vi "JYSp.vi"() -> ()   [LabVIEW 2015]
uses:
  <vilib>/Utility/file.llb/Write Delimited Spreadsheet (I64).vi
panel:
  out "画图横轴":i32[][](array[numeric])
  out "Spectrum":cluster{"Y":dbl[], "Y":dbl[]}[](graph)
  out "Data":i32[](array[numeric])
  out "Intensity Graph":dbl[][](graph)
  out "最终存储路径":path
  in  "Move To\nTarget Positions":bool
  in  "Target\nFront Entrance":dbl=1.0
  in  "Entrance Mirror":u16(ring)=2 caption="Target Position\nEntrance Mirror" items=["Front"=2, "Side"=3]
  in  "Exit Mirror":u16(ring)=3 caption="Target Position Exit Mirror" items=["Front"=2, "Side"=3]
  in  "Target WL":dbl=710.0
  out "Front Entrance":dbl
  out "Units 2":string="mm"
  out "error out":errorcluster
  out "Entrance Mirror\nPosition":i32(ring)=2 items=["EntranceMirror", "ExitMirror", "Front", "Side"]
  out "Exit Mirror\nPosition":i32(ring)=2 items=["EntranceMirror", "ExitMirror", "Front", "Side"]
  out "Current WL":dbl=897.9988
  out "Units":string="nm"
  out "Current Grating":dbl=1200.0
  out "Grating Index":i32=1
  out "Current Description":string="1" caption="Description"
  in  "Target Grating":string(combo)="2"
  out "Gratings":dbl[](array[numeric])=[1200.0, 300.0]
  in  "Force\nInitialization":bool
  out "Initialized JY":bool=TRUE
  in  "Connect":bool
  in  "Mono ID":string(combo)="Mono1"
  out "Current UniqueID":string="Mono4"
  in  "Constante de condition\n(Voir l'aide contextuelle)":bool
  out "trigAddress":i32
  in  "Commande tab":T1(tab)
  in  "Area Number to Display":i32
  in  "Reformat":bool
  in  "GAIN":u16(ring) caption="Device Name" items=["High Light", "Best Dynamic Range", "High Sensitivity"]
  in  "ADC":u16(ring) caption="Device Name" items=["20 kHz       ", " 1 MHz       ", " 1 MHz Ultra "]
  in  "Number of Areas :":u16=1 min=1 step=1
  in  "Integration time (ms) :":i16=500
  out "Uniques ID":u16(ring) items=["CCD1", "CCD2"]
  in  "Device Name":u16(ring) items=["Synapse CCD (Lateral)", "Synapse_IGA (Axial)"]
  in  "Signal type :":enum16{"TTL Rising Edge", "TTL Falling Edge"}(ring)=enum."TTL Falling Edge"
  in  "Trigger Type :":u16(ring) items=["On Start"=1, "Per Acquisition"=2]
  in  "trigSigTypeString":string
  in  "trigEventString":string
  in  "Enable InputTriggers :":bool
  in  "Number of Cleans":i32=1
  in  "MultiAcqShutterMode":i32(ring)=3 items=["Open For All Spectra"=1, "Open for Each Spectrum"=3]
  in  "Accumulations:":u16=10 min=1 step=1
  in  "Multi Accumulation mode:":bool
  out "Y Pixels:":i32=256
  out "DataSize":i32=1024
  out "X Pixels:":i32=1024
  out "Firmware\nVersion":string="V1.20 CCD_4000"
  out "Acq Time(ms)":u32=3401
  out "Gain Number":i32[](array[numeric])=[10, 11, 12, 13, 8, 2]
  out "ADC Number":i32[](array[numeric])=[0, 1, 2, 3, 4]
  out "initialized ?":bool=TRUE
  in  "Continuous":bool
  in  "CCD Busy":bool
  in  "ShutterOpen":bool=TRUE caption="Shutter enable"
  out "temp graph":dbl(graph)=-134.538067
  in  "Temperature":bool
  out "areas :":i32[][](array[numeric])=[[1], [1], [1], [1024], [256], [1], [256]]
  in  "Acquire":bool
  in  "Setup":bool
  in  "Close":bool=TRUE
  out "indicator":string="Ready !"
  in  "initialize":bool
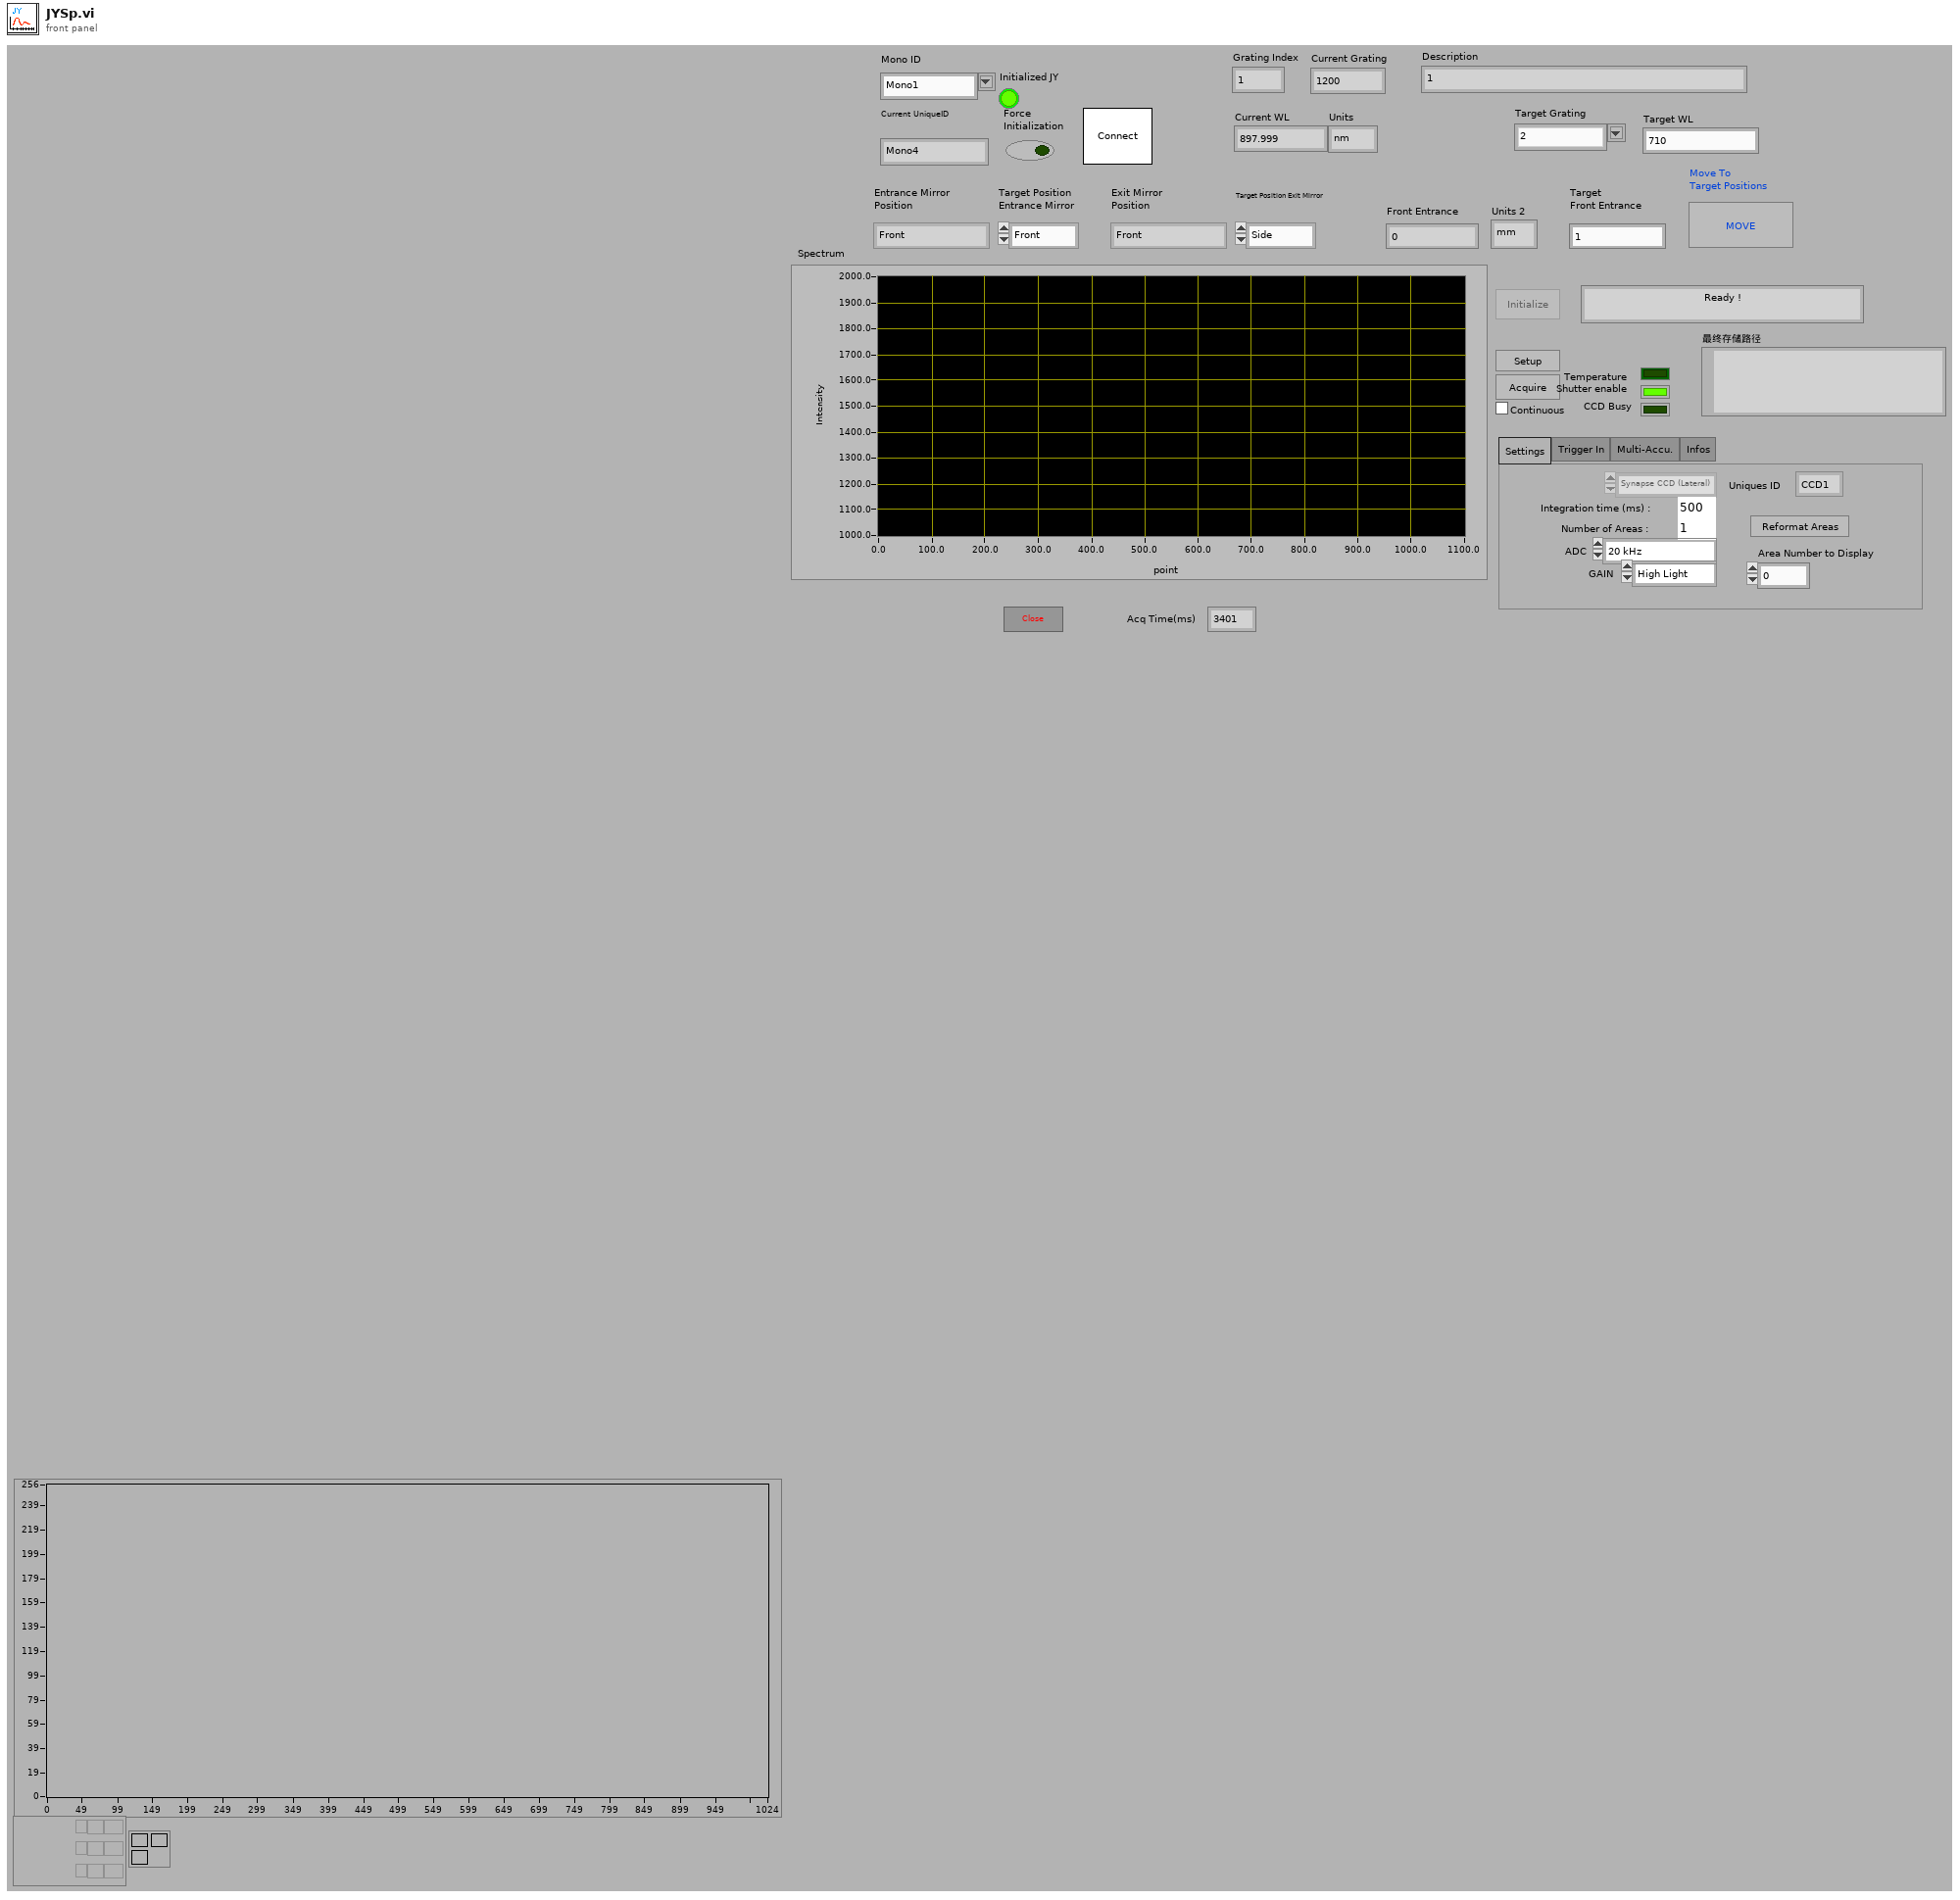
[diagram p1: front panel]
types:
  T1 = enum32{"Settings", "Trigger In", "Multi-Accu.", "Infos"}
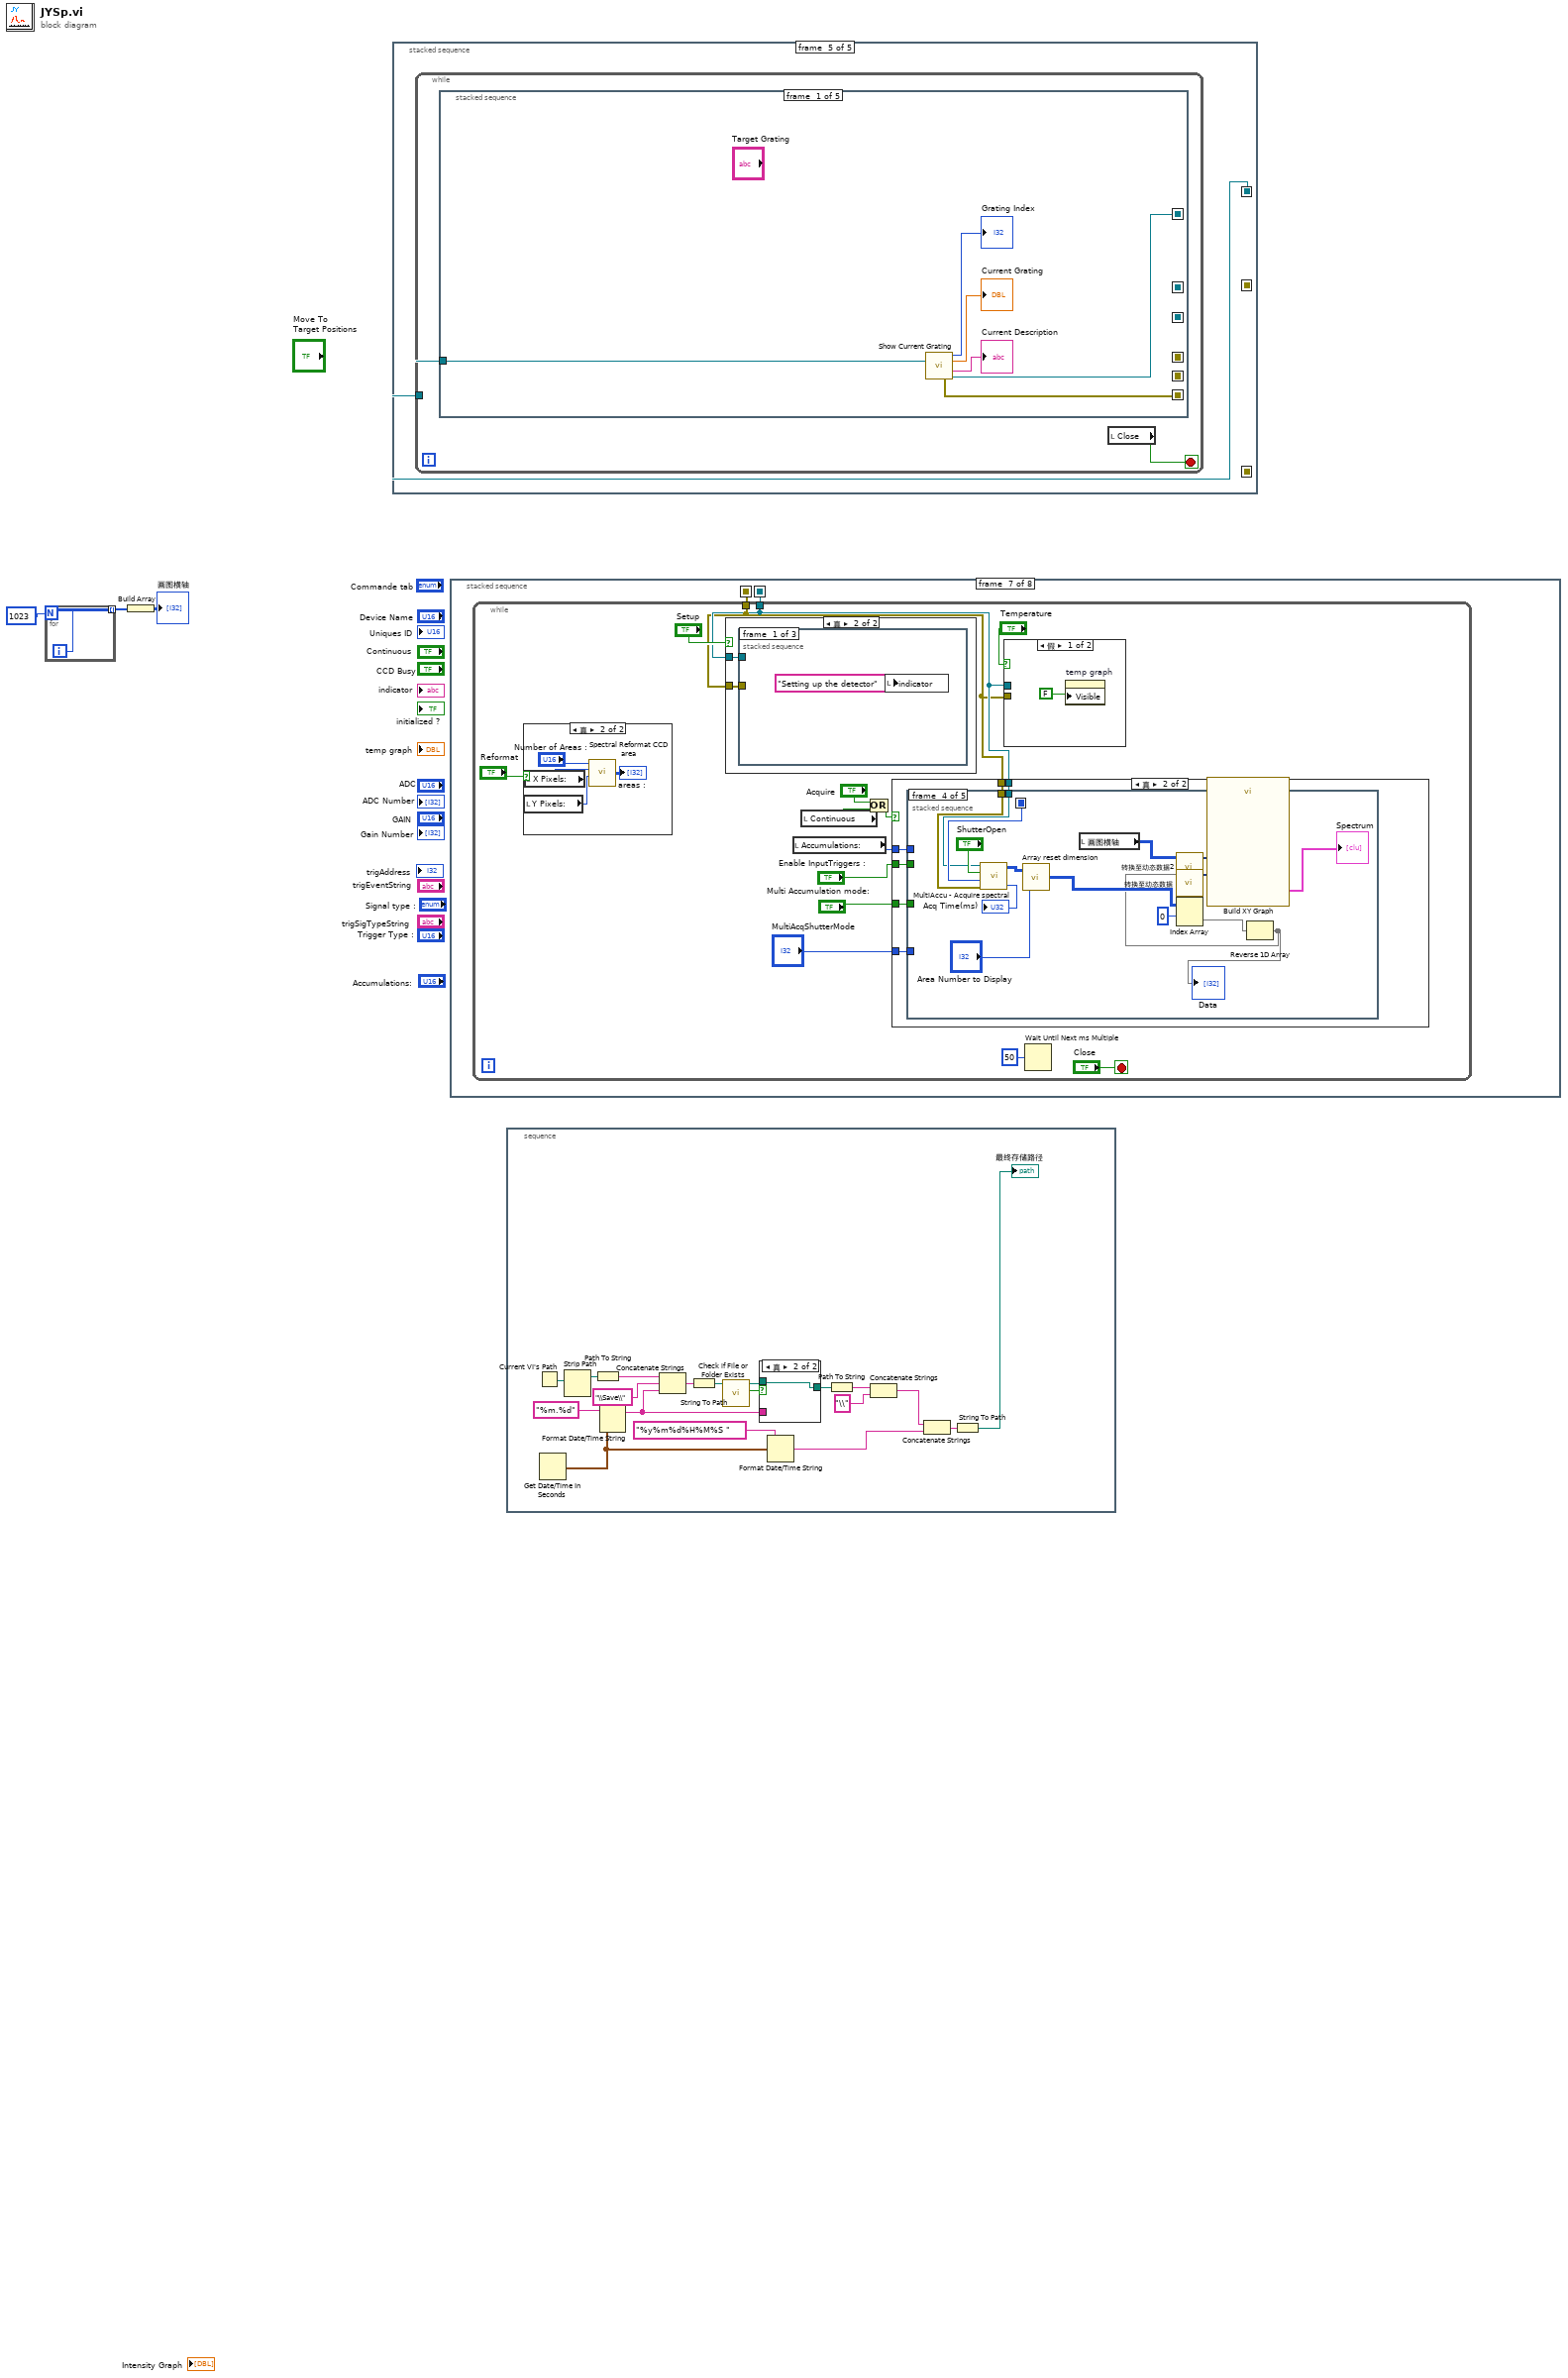
[diagram p0: block diagram]
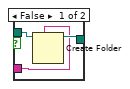
[diagram p2: hidden frame]
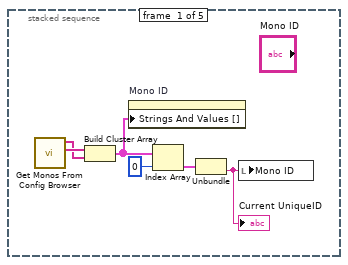
[diagram p3: hidden frame]
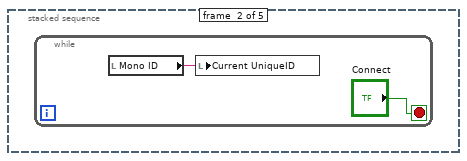
[diagram p4: hidden frame]
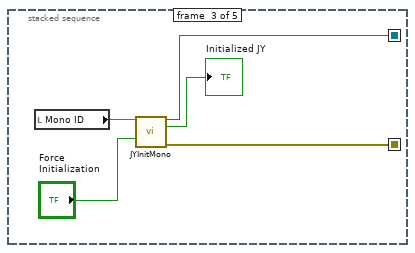
[diagram p5: hidden frame]
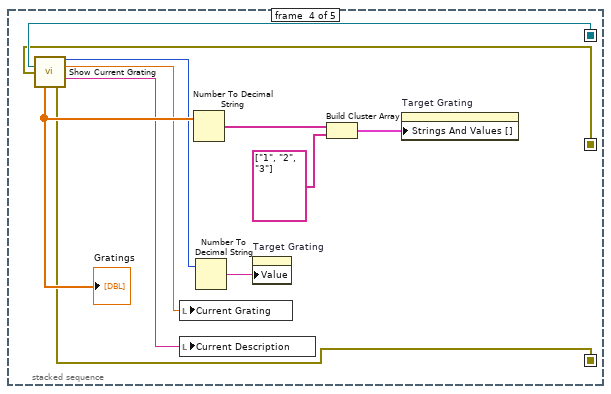
[diagram p6: hidden frame]
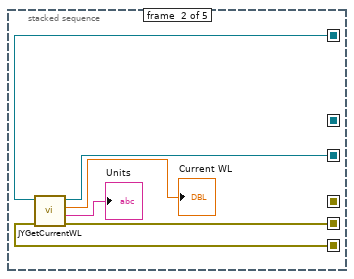
[diagram p7: hidden frame]
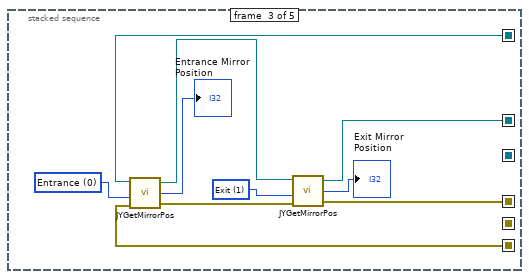
[diagram p8: hidden frame]
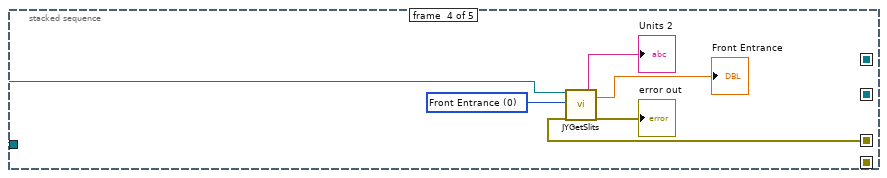
[diagram p9: hidden frame]
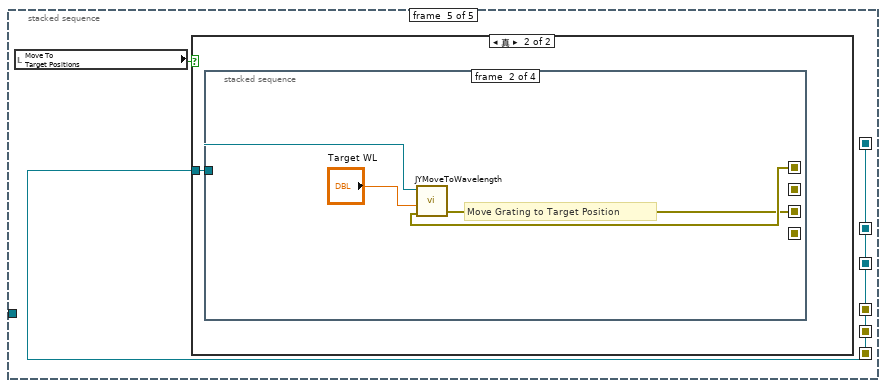
[diagram p10: hidden frame]
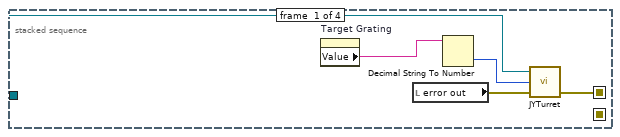
[diagram p12: hidden frame]
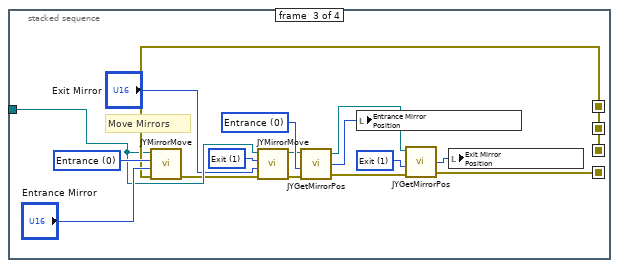
[diagram p13: hidden frame]
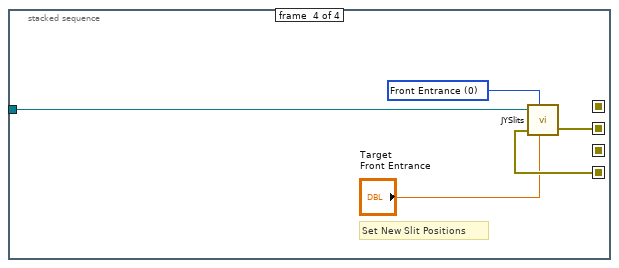
[diagram p14: hidden frame]
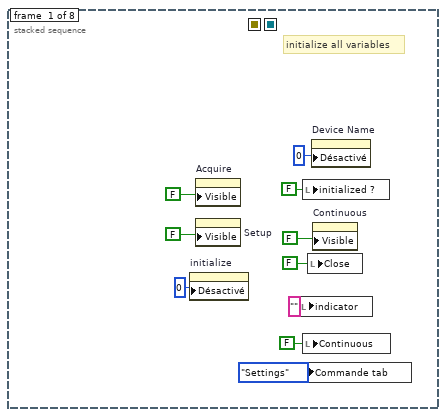
[diagram p15: hidden frame]
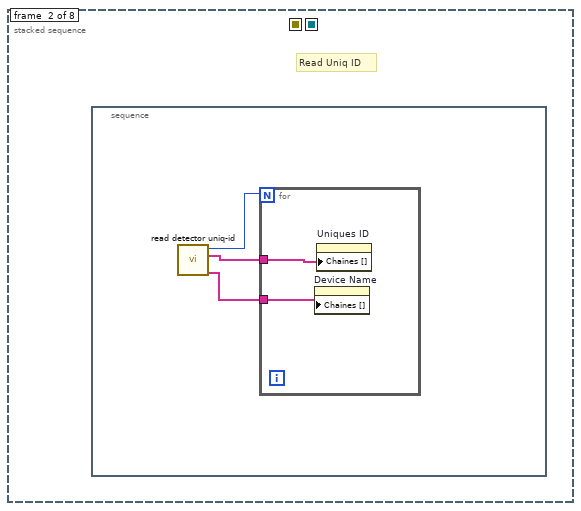
[diagram p16: hidden frame]
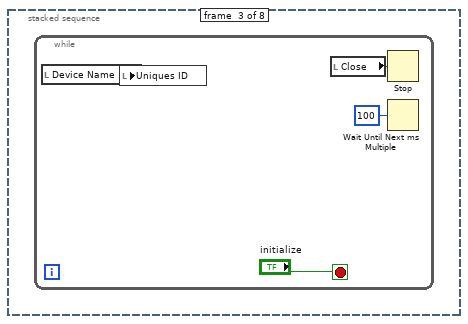
[diagram p17: hidden frame]
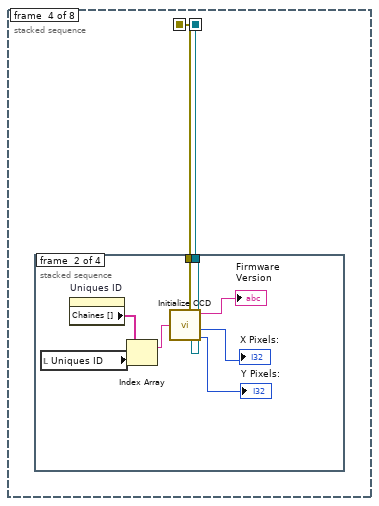
[diagram p18: hidden frame]
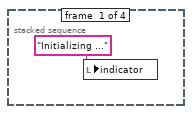
[diagram p19: hidden frame]
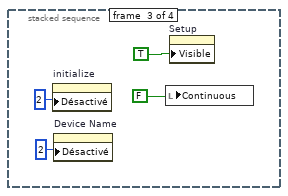
[diagram p20: hidden frame]
diagram:
  n1 = for {
    N: 1023 -> [_]
    tunnel: [w4] -> w3 mode=indexing
    i -> [w4]
  }
  n2 = Build Array(w3) -> (→"画图横轴":i32[][])
  n3 = stacked-sequence {
    seq-local: [_ _ w14 _ _] -> [_ _ _ w24 w29]
    seq-local: [_ _ w13 _ _] -> [_ _ _ w23 _]
    seq-local: [_ _ _ w22 _] -> [_ _ _ _ _]
    frame #0 {
      n4 = call "Get Monos From Config Browser.vi"() -> ("UniqueIDs"=w9:string[], "Mono ID"=w10:string[])  [unwired: 3 in, 1 out]
      n5 = Build Cluster Array(w10, w9) -> (w7:cluster{"String":string, "String":string}[])
      n6 = property on="Mono ID" class="CmbBox"("Strings And Values []"=w7) -> ()  [unwired: 2 in, 2 out]
      n7 = Index Array(array=w7, index=0) -> (element=w8:cluster{"String":string, "String":string})
      n8 = Unbundle(w8) -> ("String"=w5:string)  [unwired: 1 out]
      "Current UniqueID" <- w5
      n9 = local write "Mono ID"(w5) -> ()
    }
    frame #1 {
      n10 = while {
        stop <- "Connect" stop-if-true
        n11 = local read "Mono ID"() -> (w11:string)
        n12 = local write "Current UniqueID"(w11) -> ()
      }
    }
    frame #2 {
      n13 = local read "Mono ID"() -> (w16:string)
      n14 = call "JYInitMono.vi"("Unique ID"=w16, "Force Init"="Force\nInitialization") -> ("Refnum out"=w14:refnum<k7>, "Initialized"=→"Initialized JY":bool, "error out"=w13:errorcluster)  [unwired: 9 in, 2 out]
    }
    frame #3 {
      n15 = call "Show Current Grating.vi"("Refnum in"=w24, "error in (no error)"=w23) -> ("Gratings"=w25:dbl[], "Grating Index"=w19:i32, "Current Grating"=w21:dbl, "Current Description"=w18:string, "error out"=w22:errorcluster)  [unwired: 5 in, 4 out]
      "Gratings" <- w25
      n16 = local write "Current Grating"(w21) -> ()
      n17 = local write "Current Description"(w18) -> ()
      n18 = Number To Decimal String(number=w25) -> (decimal integer string=w27:string[])  [unwired: 1 in]
      n19 = Number To Decimal String(number=w19) -> (decimal integer string=w20:string)  [unwired: 1 in]
      n20 = property on="Target Grating" class="CmbBox"("Value"=w20) -> ()  [unwired: 2 in, 2 out]
      n21 = Build Cluster Array(w27, string[] ["1", "2", "3"]) -> (w28:cluster{"Numeric":string, string}[])
      n22 = property on="Target Grating" class="CmbBox"("Strings And Values []"=w28) -> ()  [unwired: 2 in, 2 out]
    }
    frame #4 {
      n23 = while {
        tunnel: w29 -> [w31]
        stop <- w30 stop-if-true
        n24 = stacked-sequence {
          seq-local: [w35 _ _ _ _] -> [_ w42 w53 _ w60]
          seq-local: [w34 _ _ _ _] -> [_ w41 w52 _ _]
          seq-local: [_ w40 _ _ _] -> [_ _ _ _ _]
          seq-local: [_ w39 _ _ _] -> [_ _ _ _ _]
          seq-local: [_ _ w45 _ _] -> [_ _ _ _ _]
          seq-local: [_ _ w44 _ _] -> [_ _ _ w55 _]
          tunnel: w31 -> [w33 _ _ w56 _]
          frame #0 {
            n25 = call "Show Current Grating.vi"("Refnum in"=w33) -> ("Grating Index"=→"Grating Index":i32, "Current Grating"=→"Current Grating":dbl, "Current Description"=→"Current Description":string, "error out"=w34:errorcluster, "JYMONOLib.IJYMonoReqd"=w35:refnum<k7>)  [unwired: 6 in, 4 out]
          }
          frame #1 {
            n26 = call "JYGetCurrentWL.vi"("error in (no error)"=w41, "JYMONOLib.IJYMonoReqd"=w42) -> ("error out"=w39:errorcluster, "Units"=→"Units":string, "Current WL"=→"Current WL":dbl, "JYMONOLib.IJYMonoReqd 2"=w40:refnum<k7>)  [unwired: 6 in]
          }
          frame #2 {
            w50 = u16 1 items=["Entrance", "Exit"] ("Mirror Number")
            w51 = u16 0 items=["Entrance", "Exit"] ("Mirror Number")
            n27 = call "JYGetMirrorPos.vi"("error in (no error)"=w52, "Mirror"=w51, "Refnum In"=w53) -> ("error out"=w48:errorcluster, "Current Mirror Position"=→"Entrance Mirror\nPosition":i32, "Refnum Out"=w49:refnum<k7>)  [unwired: 1 in]
            n28 = call "JYGetMirrorPos.vi"("error in (no error)"=w48, "Mirror"=w50, "Refnum In"=w49) -> ("error out"=w44:errorcluster, "Current Mirror Position"=→"Exit Mirror\nPosition":i32, "Refnum Out"=w45:refnum<k7>)  [unwired: 1 in]
          }
          frame #3 {
            w58 = u16 0 items=["Front Entrance", "Side Entrance", "Front Exit", "Side Exit", "First Intermediate", "Second Intermediate"] ("Slit")
            n29 = call "JYGetSlits.vi"("MonoRefNum IN"=w56, "Slit"=w58, "error in (no error)"=w55) -> ("Units"=→"Units 2":string, "Slit Width"=→"Front Entrance":dbl, "error out"=→"error out":errorcluster)  [unwired: 13 in, 1 out]
          }
          frame #4 {
            n30 = local read "Move To\nTarget Positions"() -> (w61:bool)
            n31 = case shown="真" w61 {
              tunnel: w60 -> [_ w62]
              frame False {
              }
              frame True {
                n32 = stacked-sequence {
                  seq-local: [w64 _ _ _] -> [_ w70 _ _]
                  seq-local: [_ w68 _ _] -> [_ _ w85 _]
                  seq-local: [_ _ w72 _] -> [_ _ _ w91]
                  seq-local: [_ _ _ w88] -> [_ _ _ _]
                  tunnel: w62 -> [w66 w69 w83 w92]
                  frame #0 {
                    n33 = property on="Target Grating" class="CmbBox"() -> ("Value"=w63:string)  [unwired: 2 in, 2 out]
                    n34 = local read "error out"() -> (w65:errorcluster)
                    n35 = Decimal String To Number(string=w63) -> (number=w67:i32)  [unwired: 2 in, 1 out]
                    n36 = call "JYTurret.vi"("error in (no error)"=w65, "Grating Index"=w67, "JYMONOLib.IJYMonoReqd"=w66) -> ("error out"=w64:errorcluster)  [unwired: 2 out]
                  }
                  frame #1 {
                    # "Move Grating to Target Position"
                    n37 = call "JYMoveToWavelength.vi"("error in (no error)"=w70, "Target WL"="Target WL", "RefNum In"=w69) -> ("error out"=w68:errorcluster)  [unwired: 1 in, 2 out]
                  }
                  frame #2 {
                    w78 = u16 1 items=["Entrance", "Exit"] ("Mirror Number")
                    w77 = u16 0 items=["Entrance", "Exit"] ("Mirror Number")
                    w84 = u16 1 items=["Entrance", "Exit", "Front", "Side"] ("Mirror Number")
                    w87 = u16 0 items=["Entrance", "Exit", "Front", "Side"] ("Mirror Number")
                    # "Move Mirrors"
                    n38 = call "JYMirrorMove.vi"("error in (no error)"=w85, "Mirror Position"="Entrance Mirror", "Mirror Number"=w87, "RefNum In"=w83) -> ("error out"=w82:errorcluster)  [unwired: 6 in, 1 out]
                    n39 = call "JYMirrorMove.vi"("error in (no error)"=w82, "Mirror Position"="Exit Mirror", "Mirror Number"=w84, "RefNum In"=w83) -> ("error out"=w75:errorcluster, "MonoRefNum Out"=w76:refnum<k7>)  [unwired: 6 in]
                    n40 = call "JYGetMirrorPos.vi"("error in (no error)"=w75, "Mirror"=w77, "Refnum In"=w76) -> ("error out"=w80:errorcluster, "Current Mirror Position"=w74:i32, "Refnum Out"=w79:refnum<k7>)  [unwired: 1 in]
                    n41 = local write "Entrance Mirror\nPosition"(w74) -> ()
                    n42 = call "JYGetMirrorPos.vi"("error in (no error)"=w80, "Mirror"=w78, "Refnum In"=w79) -> ("error out"=w72:errorcluster, "Current Mirror Position"=w73:i32)  [unwired: 1 in, 1 out]
                    n43 = local write "Exit Mirror\nPosition"(w73) -> ()
                  }
                  frame #3 {
                    w90 = u16 0 items=["Front Entrance", "Side Entrance", "Front Exit", "Side Exit", "First Intermediate", "Second Intermediate"] ("Slit")
                    # "Set New Slit Positions"
                    n44 = call "JYSlits.vi"("JYMONOLib.IJYMonoReqd"=w92, "Slit"=w90, "error in (no error)"=w91, "Slit Width"="Target\nFront Entrance") -> ("error out"=w88:errorcluster)  [unwired: 1 in, 1 out]
                  }
                }
              }
            }
          }
        }
        n45 = local read "Close"() -> (w30:bool)
      }
    }
  }
  n46 = stacked-sequence {
    seq-local: [_ _ _ w113 _ _ _ _] -> [_ _ _ _ w131 w151 w154 w266]
    seq-local: [_ _ _ w112 _ _ _ _] -> [_ _ _ _ w132 w152 w153 w267]
    frame #0 {
      # "initialize all variables"
      n47 = property on="initialize" class="Bool"("Désactivé"=u8 0) -> ()  [unwired: 2 in, 2 out]
      n48 = property on="Acquire" class="Bool"("Visible"=FALSE) -> ()  [unwired: 2 in, 2 out]
      n49 = property on="Setup" class="Bool"("Visible"=FALSE) -> ()  [unwired: 2 in, 2 out]
      n50 = local write "indicator"("" ("indicator")) -> ()
      n51 = local write "Commande tab"(T1."Settings" ("Commande tab")) -> ()
      n52 = local write "initialized ?"(FALSE ("initialized ?")) -> ()
      n53 = local write "Continuous"(FALSE ("Continuous")) -> ()
      n54 = local write "Close"(FALSE ("Close")) -> ()
      n55 = property on="Device Name" class="Ring (严格)"("Désactivé"=u8 0) -> ()  [unwired: 2 in, 2 out]
      n56 = property on="Continuous" class="Bool (严格)"("Visible"=FALSE) -> ()  [unwired: 2 in, 2 out]
    }
    frame #1 {
      # "Read Uniq ID"
      n57 = stacked-sequence {
        frame #0 {
          n58 = call <userlib>:"read detector uniq-id.vi"() -> ("nbr of components"=w105:i32, "UniqueID"=w104:string[], "Name"=w103:string[])  [unwired: 4 out]
          n59 = for {
            N: w105 -> [_]
            tunnel: w104 -> [w107]
            tunnel: w103 -> [w106]
            n60 = property on="Device Name" class="Ring (严格)"("Chaînes []"=w106) -> ()  [unwired: 2 in, 2 out]
            n61 = property on="Uniques ID" class="Ring (严格)"("Chaînes []"=w107) -> ()  [unwired: 2 in, 2 out]
          }
        }
      }
    }
    frame #2 {
      n62 = while {
        stop <- "initialize" stop-if-true
        n63 = local read "Device Name"() -> (w110:u16)
        n64 = local write "Uniques ID"(w110) -> ()
        n65 = local read "Close"() -> (w108:bool)
        n66 = Stop(stop? (T)=w108) -> ()
        n67 = Wait Until Next ms Multiple(millisecond multiple=u32 100 ("n millisecondes")) -> ()  [unwired: 1 out]
      }
    }
    frame #3 {
      n68 = stacked-sequence {
        tunnel: [_ w120 _ _] -> w113
        tunnel: [_ w119 _ _] -> w112
        frame #0 {
          n69 = local write "indicator"("Initializing ..." ("indicator")) -> ()
        }
        frame #1 {
          n70 = local read "Uniques ID"() -> (w117:u16)
          n71 = property on="Uniques ID" class="Ring (严格)"() -> ("Chaînes []"=w118:string[])  [unwired: 2 in, 2 out]
          n72 = Index Array(array=w118, index=w117) -> (element=w116:string)
          n73 = call <userlib>:"Initialize CCD.vi"("Unique id:"=w116) -> ("activeYPixels"=→"Y Pixels:":i32, "JYCCDLib.IJYCCDReqd"=w119:refnum<k7>, "activeXPixels"=→"X Pixels:":i32, "sortie d'erreur"=w120:errorcluster, "FirmwareVersion"=→"Firmware\nVersion":string)  [unwired: 3 out]
        }
        frame #2 {
          n74 = property on="initialize" class="Bool"("Désactivé"=u8 2) -> ()  [unwired: 2 in, 2 out]
          n75 = property on="Device Name" class="Ring (严格)"("Désactivé"=u8 2) -> ()  [unwired: 2 in, 2 out]
          n76 = local write "Continuous"(FALSE ("Continuous")) -> ()
          n77 = property on="Setup" class="Bool"("Visible"=TRUE) -> ()  [unwired: 2 in, 2 out]
        }
        frame #3 {
          n78 = local write "initialized ?"(TRUE ("initialized ?")) -> ()
          n79 = local write "indicator"("Initialized !" ("indicator")) -> ()
        }
      }
    }
    frame #4 {
      # "Actually not working"
      # "Read ADC and GAIN"
      n80 = case shown="真" "Constante de condition\n(Voir l'aide contextuelle)" {
        tunnel: w132 -> [_ w142]
        tunnel: w131 -> [_ w141]
        frame False {
        }
        frame True {
          # "Read Input supported trigger"
          n81 = call <userlib>:"Trigger - Get Supported Input.vi"("JYCCDLib.IJYCCDReqd"=w142, "Error Input"=w141) -> ("trigAddress"=w136:i32, "eventPtr"=w137:i32, "trigEventString"=w140:string, "trigSigType"=w139:i32, "trigSigTypeString"=w138:string)  [unwired: 4 out]
          n82 = local write "trigSigTypeString"(w138) -> ()
          n83 = local write "trigAddress"(w136) -> ()
          n84 = local write "Trigger Type :"(w137) -> ()
          n85 = local write "trigEventString"(w140) -> ()
          n86 = local write "Signal type :"(w139) -> ()
        }
      }
      n87 = call <userlib>:"Init ADC & Gain.vi"("JYCCDLib.IJYCCDReqd"=w132, "input error"=w131) -> ("ADC Number"=w130:i32[], "ADC description"=w135:string[], "Gain Number"=w133:i32[], "Gain description"=w134:string[])
      n88 = local write "Gain Number"(w133) -> ()
      n89 = local write "ADC Number"(w130) -> ()
      n90 = stacked-sequence {
        tunnel: w135 -> [w143 _]
        tunnel: w134 -> [_ w144]
        frame #0 {
          n91 = property on="ADC" class="Ring (严格)"("Chaînes []"=w143) -> ()  [unwired: 2 in, 2 out]
        }
        frame #1 {
          n92 = property on="GAIN" class="Ring (严格)"("Chaînes []"=w144) -> ()  [unwired: 2 in, 2 out]
        }
      }
    }
    frame #5 {
      # "IS multi Accumulation Supported ?"
      n93 = call <userlib>:"MultiAccu - Is Supported.vi"("Error In"=w151, "JYCCDLib.IJYCCDReqd"=w152) -> ("IsOperatingModeSupported"=w145:bool)  [unwired: 3 out]
      n94 = Select(t=0, s=w145, f=2) -> (s? t:f=w148:i32)
      n95 = Select(t=FALSE, s=w145, f=w145) -> (s? t:f=w147:bool)
      n96 = local write "Multi Accumulation mode:"(w147) -> ()
      n97 = property on="Multi Accumulation" class="Bool (严格)"("Désactivé"=w148) -> ()  [unwired: 2 in, 2 out]
      n98 = property on="Multi Accumulation mode:" class="Bool (严格)"("Désactivé"=w148) -> ()  [unwired: 2 in, 2 out]
    }
    frame #6 {
      n99 = while {
        tunnel: w153 -> [w161]
        tunnel: w154 -> [w160]
        stop <- "Close" stop-if-true
        n100 = case shown="真" "Reformat" {
          frame False {
          }
          frame True {
            n101 = local read "Y Pixels:"() -> (w244:i32)
            n102 = local read "X Pixels:"() -> (w246:i32)
            n103 = call <userlib>:"Spectral Reformat CCD area.vi"("Y Pixels:"=w244, "X Pixels:"=w246, "numAreas"="Number of Areas :") -> ("areas :"=→"areas :":i32[][])  [unwired: 3 out]
          }
        }
        n104 = case shown="真" "Setup" {
          tunnel: w160 -> [_ w249]
          tunnel: w161 -> [_ w248]
          frame False {
          }
          frame True {
            n105 = stacked-sequence {
              tunnel: w249 -> [_ w263 _]
              tunnel: w248 -> [_ w260 _]
              frame #0 {
                n106 = local write "indicator"("Setting up the detector" ("indicator")) -> ()
              }
              frame #1 {
                w261 = 1 items=["JYMCD_ACQ_FORMAT_IMAGE", "JYMCD_ACQ_FORMAT_SCAN"] ("Acquisition type")
                n107 = local read "Gain Number"() -> (w255:i32[])
                n108 = local read "GAIN"() -> (w251:u16)
                n109 = local read "ADC Number"() -> (w256:i32[])
                n110 = local read "ADC"() -> (w252:u16)
                n111 = Index Array(array=w255, index=w251) -> (element=w253:i32)
                n112 = Index Array(array=w256, index=w252) -> (element=w254:i32)
                n113 = local read "Number of Areas :"() -> (w258:u16)
                n114 = local read "areas :"() -> (w259:i32[][])
                n115 = call <userlib>:"Setup CCD.vi"("numAreas"=w258, "areas :"=w259, "JYCCDLib.IJYCCDReqd"=w260, "entrée d'erreur (pas d'erreur)"=w263, "Acquisition type"=w261, "Gain"=w253, "Select ADC"=w254, "Integration time(ms)"="Integration time (ms) :") -> ("DataSize"=→"DataSize":i32)  [unwired: 1 out]
              }
              frame #2 {
                w264 = TRUE ("Visible")
                n116 = property on="Continuous" class="Bool (严格)"("Visible"=w264) -> ()  [unwired: 2 in, 2 out]
                n117 = property on="Acquire" class="Bool"("Visible"=w264) -> ()  [unwired: 2 in, 2 out]
                n118 = local write "indicator"("Ready !" ("indicator")) -> ()
              }
            }
          }
        }
        n119 = local read "Accumulations:"() -> (w157:u16)
        n120 = local read "Continuous"() -> (w162:bool)
        n121 = Or(x="Acquire", y=w162) -> (x .or. y?=w159:bool)
        n122 = case shown="真" w159 {
          tunnel: w161 -> [_ w174]
          tunnel: w160 -> [_ w173]
          tunnel: "Enable InputTriggers :" -> [_ w172]
          tunnel: "Multi Accumulation mode:" -> [_ w171]
          tunnel: w157 -> [_ w170]
          tunnel: "MultiAcqShutterMode" -> [_ w169]
          frame False {
          }
          frame True {
            n123 = stacked-sequence {
              seq-local: [_ _ w187 _ _] -> [_ _ _ w213 _]
              tunnel: w174 -> [_ w176 w191 w212 _]
              tunnel: w173 -> [_ w177 w190 w211 _]
              tunnel: w172 -> [_ w178 _ _ _]
              tunnel: w171 -> [_ _ w189 _ _]
              tunnel: w170 -> [_ _ w188 _ _]
              tunnel: w169 -> [_ _ w186 _ _]
              frame #0 {
                n124 = local write "CCD Busy"(TRUE ("CCD Busy")) -> ()
              }
              frame #1 {
                n125 = case shown="真" w178 {
                  tunnel: w177 -> [w179 w185]
                  tunnel: w176 -> [w180 w184]
                  frame False {
                    n126 = call <userlib>:"Trigger - Disable.vi"("Error In"=w179, "JYCCDLib.IJYCCDReqd"=w180) -> ()  [unwired: 6 out]
                  }
                  frame True {
                    n127 = local read "Trigger Type :"() -> (w181:u16)
                    n128 = local read "Signal type :"() -> (w182:enum16{"TTL Rising Edge", "TTL Falling Edge"})
                    n129 = local read "trigAddress"() -> (w183:i32)
                    n130 = call <userlib>:"Trigger - Enable.vi"("Error In"=w185, "sigType"=w182, "event"=w181, "trigAddress"=w183, "JYCCDLib.IJYCCDReqd"=w184) -> ()  [unwired: 3 out]
                  }
                }
              }
              frame #2 {
                n131 = case shown="真" w189 {
                  selector: w189 -> [_ w197]
                  tunnel: w191 -> [w194 w200]
                  tunnel: w190 -> [w193 w199]
                  tunnel: w188 -> [_ w198]
                  tunnel: [u16 1 ("Accumulations:") w198] -> w187
                  tunnel: w186 -> [_ w196]
                  frame False {
                    n132 = call <userlib>:"MultiAccu - Disable.vi"("Error In"=w193, "JYCCDLib.IJYCCDReqd"=w194) -> ()  [unwired: 4 out]
                  }
                  frame True {
                    n133 = call <userlib>:"MultiAccu - Configure.vi"("JYCCDLib.IJYCCDReqd"=w200, "Cleans Before"="Number of Cleans", "Accumulations:"=w198, "MultiAcqHardwareMode"=w197, "MultiAcqShutterMode"=w196, "Error In"=w199) -> ()  [unwired: 1 in, 9 out]
                  }
                }
              }
              frame #3 {
                n134 = call <userlib>:"MultiAccu - Acquire spectral.vi"("error in"=w211, "Accumulations:"=w213, "ShutterOpen"="ShutterOpen", "JYCCDLib.IJYCCDReqd"=w212) -> ("Acq Time(ms)"=→"Acq Time(ms)":u32, "Array Out"=w210:i32[][][])  [unwired: 1 out]
                n135 = call <userlib>:"Array reset dimension.vi"("Area Number"="Area Number to Display", "Array In"=w210) -> ("Array Out"=w206:i32[][])
                n136 = local read "画图横轴"() -> (w202:i32[][])
                n137 = call "转换至动态数据2"("2D Array"=w202) -> ("Dynamic Data Type"=w201:dynamicdata)  [unwired: 3 in]
                n138 = Index Array(array=w206, index (row)=0 ("索引 (行)")) -> (element=w207:i32[])  [unwired: 1 in]
                n139 = Reverse 1D Array(array=w207) -> (reversed array=w204:i32[])
                "Data" <- w204
                n140 = call "转换至动态数据"("Array"=w204) -> ("Dynamic Data Type"=w203:dynamicdata)  [unwired: 3 in]
                n141 = call "Build XY Graph"("Y Input"=w203, "X Input"=w201) -> ("XY Graph"=→"Spectrum":cluster{"Y":dbl[], "Y":dbl[]}[])  [unwired: 8 in, 1 out]
              }
              frame #4 {
                n142 = Get Date/Time In Seconds() -> (seconds since 1Jan1904=w227:timestamp)
                n143 = local read "最终存储路径"() -> (w218:path)
                n144 = Get Date/Time String(date format (0)=enum16{"short", "long", "abbreviated"}."abbreviated" ("日期格式(0)"), seconds (now)=w227, want seconds? (F)=TRUE ("需要秒？(F)")) -> (date string=w219:string, time string=w224:string)
                n145 = local write "CCD Busy"(FALSE ("CCD Busy")) -> ()
                n146 = Search and Replace String(replace all?=TRUE ("替换全部？(F)"), input string=w224, search string=":" ("搜索字符串"), replace string="-" ("替换字符串(\"\")")) -> (result string=w220:string)  [unwired: 4 in, 3 out]
                n147 = Path To String(path=w218) -> (string=w217:string)
                n148 = Concatenate Strings(w217, w219, w220, "光谱" ("字符串"), ".xls" ("字符串")) -> (w234:string)
                n149 = String To Path(string=w234) -> (path=w230:path)
                n150 = local read "Data"() -> (w216:i32[])
                n151 = call-poly <vilib>:"Write Delimited Spreadsheet.vi"("file path (dialog if empty)"=w230, "format (%d)"="%.16f" ("format (%.3f)"), "1D data"=w216, "append to file? (F)"=TRUE, "transpose? (F)"=TRUE) -> ()  [unwired: 9 in, 2 out]
              }
            }
          }
        }
        n152 = case shown="假" "Temperature" {
          tunnel: w161 -> [_ w238]
          tunnel: w160 -> [_ w237]
          frame False {
            n153 = property on="temp graph" class="WFChart (严格)"("Visible"=FALSE) -> ()  [unwired: 2 in, 2 out]
          }
          frame True {
            n154 = stacked-sequence {
              tunnel: w238 -> [_ w243]
              tunnel: w237 -> [_ w242]
              frame #0 {
                n155 = property on="temp graph" class="WFChart (严格)"("Visible"=TRUE) -> ()  [unwired: 2 in, 2 out]
              }
              frame #1 {
                w241 = u16 0 items=["° Celsius", "Kelvin", "° Farenheit"] ("units")
                n156 = call <userlib>:"read temperature.vi"("entrée d'erreur (pas d'erreur)"=w242, "units"=w241, "JYCCDLib.IJYCCDReqd"=w243) -> ("Current Temperature"=w240:dbl)
                n157 = local write "temp graph"(w240) -> ()
              }
            }
          }
        }
        n158 = Wait Until Next ms Multiple(millisecond multiple=u32 50 ("n millisecondes")) -> ()  [unwired: 1 out]
      }
    }
    frame #7 {
      n159 = Close Reference(reference=w267, error in (no error)=w266) -> ()  [unwired: 1 out]
    }
  }
  n160 = stacked-sequence {
    frame #0 {
      n161 = Current VI's Path() -> (path=w284:path)
      n162 = Get Date/Time In Seconds() -> (seconds since 1Jan1904=w281:timestamp)
      n163 = Strip Path(path=w284) -> (stripped path=w283:path)  [unwired: 1 out]
      n164 = Path To String(path=w283) -> (string=w280:string)
      n165 = Format Date/Time String(time format string (%c)="%m.%d" ("时间格式字符串(%c)"), seconds (now)=w281) -> (date/time string=w273:string)  [unwired: 1 in]
      n166 = Concatenate Strings(w280, "\\Save\\" ("字符串"), w273) -> (w278:string)
      n167 = String To Path(string=w278) -> (path=w277:path)
      n168 = call <vilib>:"Check if File or Folder Exists.vi"("path"=w277) -> ("file or folder exists?"=w276:bool, "dup path"=w274:path)  [unwired: 8 in, 1 out]
      n169 = case shown="真" w276 {
        tunnel: [w289 w290] -> w275
        tunnel: w274 -> [w288 w290]
        tunnel: w273 -> [w287 _]
        frame False {
          n170 = Create Folder(prompt (Create Folder)=w287, path (use dialog)=w288) -> (created path=w289:path)  [unwired: 1 in, 2 out]
        }
        frame True {
        }
      }
      n171 = Format Date/Time String(time format string (%c)="%y%m%d%H%M%S " ("时间格式字符串(%c)"), seconds (now)=w281) -> (date/time string=w269:string)  [unwired: 1 in]
      n172 = Path To String(path=w275) -> (string=w272:string)
      n173 = Concatenate Strings(w272, "\\" ("字符串")) -> (w270:string)
      n174 = Concatenate Strings(w270, w269) -> (w286:string)
      n175 = String To Path(string=w286) -> (path=→"最终存储路径":path)
    }
  }
